vi "RemoteVI Post Menu Key.vi"(0 "hWnd":u64, 5 "vk":u64, 7 "key lParam":i64=1, 11 "error in":errorcluster) -> (15 "error out":errorcluster)   [LabVIEW 2020, in "RemoteVI.lvlib"]
doc: "Drives an open LabVIEW menu with one key: posts WM_KEYDOWN and WM_KEYUP of vk (lParam key lParam - repeat count 1, the key's scan code and the extended bit - plus the previous-state and transition bits 0xC0000000 for the key-up) to hWnd, the served panel, with user32 PostMessageW, then waits until LabVIEW has handled them (RemoteVI Wait Input Handled.vi, two WM_NULL sent - handled inside the menu's modal loop too). LabVIEW menus take posted keys from the panel window while the menu is open, also while a submenu is open, and paint the result before that wait returns (measured on LabVIEW 2025: VK_DOWN/VK_UP move the highlight by one item, skipping separators, and wrap around at the ends; VK_RIGHT opens the highlighted item's submenu next to its parent; VK_RETURN chooses the highlighted item or opens its submenu; VK_LEFT closes the deepest submenu; a custom popup such as the colour picker takes no keys). Used by RemoteVI Highlight Menu Row.vi, RemoteVI Menu Click.vi and RemoteVI Menu Hover.vi. Win32 only, no VI Server call, so it runs while the menu's modal loop holds LabVIEW's UI thread. An incoming error posts nothing."
uses:
  RemoteVI.lvlib
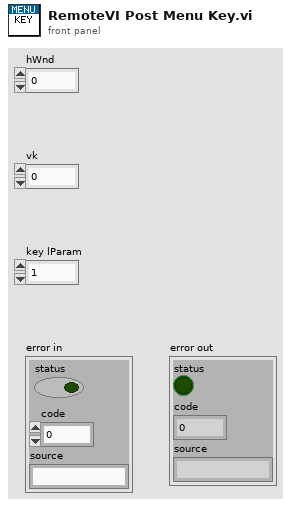
[diagram p1: front panel]
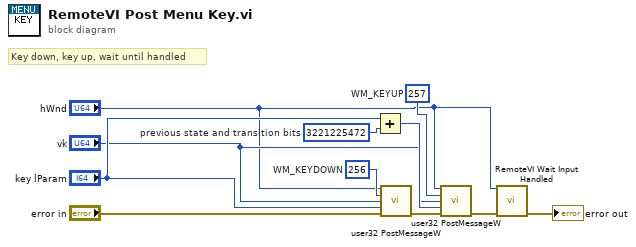
[diagram p0: block diagram]
diagram:
  w7 = i64 3221225472  # previous state and transition bits
  w6 = u32 257  # WM_KEYUP
  w5 = u32 256  # WM_KEYDOWN
  # "Key down, key up, wait until handled"
  n1 = Add(x="key lParam", y=w7) -> (x+y=w8:i64)
  n2 = call "user32 PostMessageW.vi"("hWnd"="hWnd", "Msg"=w5, "wParam"="vk", "lParam"="key lParam", "error in (no error)"="error in") -> ("error out"=w9:errorcluster)  [unwired: 9 in, 1 out]
  n3 = call "user32 PostMessageW.vi"("hWnd"="hWnd", "Msg"=w6, "wParam"="vk", "lParam"=w8, "error in (no error)"=w9) -> ("error out"=w10:errorcluster)  [unwired: 9 in, 1 out]
  n4 = call "RemoteVI Wait Input Handled.vi"("hWnd"="hWnd", "error in"=w10) -> ("error out"=→"error out":errorcluster)  [unwired: 13 in]
